vi "Integer Representation Test.vi"() -> ()   [LabVIEW 2026, in "Utility.lvlib"]
uses:
  Utility.lvlib
  Types/Signed Representation.ctl
  913b890a-b0f4-4715-82c4-53c9b125f797.vi
  de269a94-3f4e-4f39-b3db-9fb101915407.vi
  9b4d6897-da67-4ca5-9ae3-ea53d4320284.vi
  3e9a7e41-c2e1-426e-9bc1-8a394e217d85.vi
  1327767c-dc11-4062-be7d-752ab4d70a8a.vi
  1d7e0380-15ec-4017-ad21-249a48283e6f.vi
  7fe95ae4-1eaf-41d9-8065-e14043517ae9.vi
  1beec93f-fbc7-42dc-88dc-d3ecba0fc0bd.vi
  913b890a-b0f4-4715-82c4-53c9b125f797.vi/fdd2035b-52a6-4314-93d5-e6d0012ea0d5.vi
  913b890a-b0f4-4715-82c4-53c9b125f797.vi/d7ddfa2c-0539-47bf-9b9d-3a470632982d.vi
  913b890a-b0f4-4715-82c4-53c9b125f797.vi/b8120071-ec88-4802-9c07-9d147ec9c255.vi
  913b890a-b0f4-4715-82c4-53c9b125f797.vi/96d3ddf9-193f-4353-8b9f-7b29ff2119cb.vi
  913b890a-b0f4-4715-82c4-53c9b125f797.vi/a2043324-c5a4-4327-a6d6-ab77c0f4b7eb.vi
  de269a94-3f4e-4f39-b3db-9fb101915407.vi/075529c4-3756-4c35-a727-d79a570b4e4b.vi
  de269a94-3f4e-4f39-b3db-9fb101915407.vi/f2b159a7-3f15-4c07-8087-86d897f3e084.vi
  de269a94-3f4e-4f39-b3db-9fb101915407.vi/e7f4747e-5a28-4a2e-9592-f11bd74c8d05.vi
  de269a94-3f4e-4f39-b3db-9fb101915407.vi/dfb42b1f-79ab-4f7c-b389-1108b947dcfb.vi
  de269a94-3f4e-4f39-b3db-9fb101915407.vi/5f52ec6b-8d9c-4a1b-8cba-4e2f2acbbc65.vi
  de269a94-3f4e-4f39-b3db-9fb101915407.vi/9402299f-8d08-4b56-b955-c752433d99a7.vi
  de269a94-3f4e-4f39-b3db-9fb101915407.vi/587ca7da-2917-4b98-b856-e292118fa9d0.vi
  de269a94-3f4e-4f39-b3db-9fb101915407.vi/d9cf77ad-bfa9-4690-bb58-8188d63c027f.vi
  de269a94-3f4e-4f39-b3db-9fb101915407.vi/0dbe1b4e-815d-48eb-bf8e-9c4112dc030e.vi
  9b4d6897-da67-4ca5-9ae3-ea53d4320284.vi/fdd2035b-52a6-4314-93d5-e6d0012ea0d5.vi
  9b4d6897-da67-4ca5-9ae3-ea53d4320284.vi/d7ddfa2c-0539-47bf-9b9d-3a470632982d.vi
  9b4d6897-da67-4ca5-9ae3-ea53d4320284.vi/b8120071-ec88-4802-9c07-9d147ec9c255.vi
  9b4d6897-da67-4ca5-9ae3-ea53d4320284.vi/96d3ddf9-193f-4353-8b9f-7b29ff2119cb.vi
  9b4d6897-da67-4ca5-9ae3-ea53d4320284.vi/a2043324-c5a4-4327-a6d6-ab77c0f4b7eb.vi
  3e9a7e41-c2e1-426e-9bc1-8a394e217d85.vi/075529c4-3756-4c35-a727-d79a570b4e4b.vi
  3e9a7e41-c2e1-426e-9bc1-8a394e217d85.vi/f2b159a7-3f15-4c07-8087-86d897f3e084.vi
  3e9a7e41-c2e1-426e-9bc1-8a394e217d85.vi/e7f4747e-5a28-4a2e-9592-f11bd74c8d05.vi
  3e9a7e41-c2e1-426e-9bc1-8a394e217d85.vi/dfb42b1f-79ab-4f7c-b389-1108b947dcfb.vi
  3e9a7e41-c2e1-426e-9bc1-8a394e217d85.vi/5f52ec6b-8d9c-4a1b-8cba-4e2f2acbbc65.vi
  3e9a7e41-c2e1-426e-9bc1-8a394e217d85.vi/9402299f-8d08-4b56-b955-c752433d99a7.vi
  3e9a7e41-c2e1-426e-9bc1-8a394e217d85.vi/587ca7da-2917-4b98-b856-e292118fa9d0.vi
  3e9a7e41-c2e1-426e-9bc1-8a394e217d85.vi/d9cf77ad-bfa9-4690-bb58-8188d63c027f.vi
  3e9a7e41-c2e1-426e-9bc1-8a394e217d85.vi/0dbe1b4e-815d-48eb-bf8e-9c4112dc030e.vi
  1327767c-dc11-4062-be7d-752ab4d70a8a.vi/fdd2035b-52a6-4314-93d5-e6d0012ea0d5.vi
  1327767c-dc11-4062-be7d-752ab4d70a8a.vi/d7ddfa2c-0539-47bf-9b9d-3a470632982d.vi
  1327767c-dc11-4062-be7d-752ab4d70a8a.vi/b8120071-ec88-4802-9c07-9d147ec9c255.vi
  1327767c-dc11-4062-be7d-752ab4d70a8a.vi/96d3ddf9-193f-4353-8b9f-7b29ff2119cb.vi
  1327767c-dc11-4062-be7d-752ab4d70a8a.vi/a2043324-c5a4-4327-a6d6-ab77c0f4b7eb.vi
  1d7e0380-15ec-4017-ad21-249a48283e6f.vi/075529c4-3756-4c35-a727-d79a570b4e4b.vi
  1d7e0380-15ec-4017-ad21-249a48283e6f.vi/f2b159a7-3f15-4c07-8087-86d897f3e084.vi
  1d7e0380-15ec-4017-ad21-249a48283e6f.vi/e7f4747e-5a28-4a2e-9592-f11bd74c8d05.vi
  1d7e0380-15ec-4017-ad21-249a48283e6f.vi/dfb42b1f-79ab-4f7c-b389-1108b947dcfb.vi
  1d7e0380-15ec-4017-ad21-249a48283e6f.vi/5f52ec6b-8d9c-4a1b-8cba-4e2f2acbbc65.vi
  1d7e0380-15ec-4017-ad21-249a48283e6f.vi/9402299f-8d08-4b56-b955-c752433d99a7.vi
  1d7e0380-15ec-4017-ad21-249a48283e6f.vi/587ca7da-2917-4b98-b856-e292118fa9d0.vi
  1d7e0380-15ec-4017-ad21-249a48283e6f.vi/d9cf77ad-bfa9-4690-bb58-8188d63c027f.vi
  1d7e0380-15ec-4017-ad21-249a48283e6f.vi/0dbe1b4e-815d-48eb-bf8e-9c4112dc030e.vi
  7fe95ae4-1eaf-41d9-8065-e14043517ae9.vi/fdd2035b-52a6-4314-93d5-e6d0012ea0d5.vi
  7fe95ae4-1eaf-41d9-8065-e14043517ae9.vi/d7ddfa2c-0539-47bf-9b9d-3a470632982d.vi
  7fe95ae4-1eaf-41d9-8065-e14043517ae9.vi/b8120071-ec88-4802-9c07-9d147ec9c255.vi
  7fe95ae4-1eaf-41d9-8065-e14043517ae9.vi/96d3ddf9-193f-4353-8b9f-7b29ff2119cb.vi
  7fe95ae4-1eaf-41d9-8065-e14043517ae9.vi/a2043324-c5a4-4327-a6d6-ab77c0f4b7eb.vi
  1beec93f-fbc7-42dc-88dc-d3ecba0fc0bd.vi/075529c4-3756-4c35-a727-d79a570b4e4b.vi
  1beec93f-fbc7-42dc-88dc-d3ecba0fc0bd.vi/f2b159a7-3f15-4c07-8087-86d897f3e084.vi
  1beec93f-fbc7-42dc-88dc-d3ecba0fc0bd.vi/e7f4747e-5a28-4a2e-9592-f11bd74c8d05.vi
  1beec93f-fbc7-42dc-88dc-d3ecba0fc0bd.vi/dfb42b1f-79ab-4f7c-b389-1108b947dcfb.vi
  1beec93f-fbc7-42dc-88dc-d3ecba0fc0bd.vi/5f52ec6b-8d9c-4a1b-8cba-4e2f2acbbc65.vi
  1beec93f-fbc7-42dc-88dc-d3ecba0fc0bd.vi/9402299f-8d08-4b56-b955-c752433d99a7.vi
  1beec93f-fbc7-42dc-88dc-d3ecba0fc0bd.vi/587ca7da-2917-4b98-b856-e292118fa9d0.vi
  1beec93f-fbc7-42dc-88dc-d3ecba0fc0bd.vi/d9cf77ad-bfa9-4690-bb58-8188d63c027f.vi
  1beec93f-fbc7-42dc-88dc-d3ecba0fc0bd.vi/0dbe1b4e-815d-48eb-bf8e-9c4112dc030e.vi
  913b890a-b0f4-4715-82c4-53c9b125f797.vi/b8120071-ec88-4802-9c07-9d147ec9c255.vi/8ccb98a6-deb9-4b5a-be05-054c1c212d54.vi
  913b890a-b0f4-4715-82c4-53c9b125f797.vi/b8120071-ec88-4802-9c07-9d147ec9c255.vi/f171c548-4dcc-4c0c-949b-fc0df33543c2.vi
  913b890a-b0f4-4715-82c4-53c9b125f797.vi/b8120071-ec88-4802-9c07-9d147ec9c255.vi/d8adcdbd-60f3-48f3-8f6a-253ba0c2f91d.vi
  913b890a-b0f4-4715-82c4-53c9b125f797.vi/b8120071-ec88-4802-9c07-9d147ec9c255.vi/e61c01d5-f4be-4974-af39-63853a8697d8.vi
  913b890a-b0f4-4715-82c4-53c9b125f797.vi/96d3ddf9-193f-4353-8b9f-7b29ff2119cb.vi/8ccb98a6-deb9-4b5a-be05-054c1c212d54.vi
  913b890a-b0f4-4715-82c4-53c9b125f797.vi/96d3ddf9-193f-4353-8b9f-7b29ff2119cb.vi/f171c548-4dcc-4c0c-949b-fc0df33543c2.vi
  913b890a-b0f4-4715-82c4-53c9b125f797.vi/96d3ddf9-193f-4353-8b9f-7b29ff2119cb.vi/d8adcdbd-60f3-48f3-8f6a-253ba0c2f91d.vi
  913b890a-b0f4-4715-82c4-53c9b125f797.vi/96d3ddf9-193f-4353-8b9f-7b29ff2119cb.vi/e61c01d5-f4be-4974-af39-63853a8697d8.vi
  9b4d6897-da67-4ca5-9ae3-ea53d4320284.vi/b8120071-ec88-4802-9c07-9d147ec9c255.vi/8ccb98a6-deb9-4b5a-be05-054c1c212d54.vi
  9b4d6897-da67-4ca5-9ae3-ea53d4320284.vi/b8120071-ec88-4802-9c07-9d147ec9c255.vi/f171c548-4dcc-4c0c-949b-fc0df33543c2.vi
  9b4d6897-da67-4ca5-9ae3-ea53d4320284.vi/b8120071-ec88-4802-9c07-9d147ec9c255.vi/d8adcdbd-60f3-48f3-8f6a-253ba0c2f91d.vi
  9b4d6897-da67-4ca5-9ae3-ea53d4320284.vi/b8120071-ec88-4802-9c07-9d147ec9c255.vi/e61c01d5-f4be-4974-af39-63853a8697d8.vi
  9b4d6897-da67-4ca5-9ae3-ea53d4320284.vi/96d3ddf9-193f-4353-8b9f-7b29ff2119cb.vi/8ccb98a6-deb9-4b5a-be05-054c1c212d54.vi
  9b4d6897-da67-4ca5-9ae3-ea53d4320284.vi/96d3ddf9-193f-4353-8b9f-7b29ff2119cb.vi/f171c548-4dcc-4c0c-949b-fc0df33543c2.vi
  9b4d6897-da67-4ca5-9ae3-ea53d4320284.vi/96d3ddf9-193f-4353-8b9f-7b29ff2119cb.vi/d8adcdbd-60f3-48f3-8f6a-253ba0c2f91d.vi
  9b4d6897-da67-4ca5-9ae3-ea53d4320284.vi/96d3ddf9-193f-4353-8b9f-7b29ff2119cb.vi/e61c01d5-f4be-4974-af39-63853a8697d8.vi
  1327767c-dc11-4062-be7d-752ab4d70a8a.vi/b8120071-ec88-4802-9c07-9d147ec9c255.vi/8ccb98a6-deb9-4b5a-be05-054c1c212d54.vi
  1327767c-dc11-4062-be7d-752ab4d70a8a.vi/b8120071-ec88-4802-9c07-9d147ec9c255.vi/f171c548-4dcc-4c0c-949b-fc0df33543c2.vi
  1327767c-dc11-4062-be7d-752ab4d70a8a.vi/b8120071-ec88-4802-9c07-9d147ec9c255.vi/d8adcdbd-60f3-48f3-8f6a-253ba0c2f91d.vi
  1327767c-dc11-4062-be7d-752ab4d70a8a.vi/b8120071-ec88-4802-9c07-9d147ec9c255.vi/e61c01d5-f4be-4974-af39-63853a8697d8.vi
  1327767c-dc11-4062-be7d-752ab4d70a8a.vi/96d3ddf9-193f-4353-8b9f-7b29ff2119cb.vi/8ccb98a6-deb9-4b5a-be05-054c1c212d54.vi
  1327767c-dc11-4062-be7d-752ab4d70a8a.vi/96d3ddf9-193f-4353-8b9f-7b29ff2119cb.vi/f171c548-4dcc-4c0c-949b-fc0df33543c2.vi
  1327767c-dc11-4062-be7d-752ab4d70a8a.vi/96d3ddf9-193f-4353-8b9f-7b29ff2119cb.vi/d8adcdbd-60f3-48f3-8f6a-253ba0c2f91d.vi
  1327767c-dc11-4062-be7d-752ab4d70a8a.vi/96d3ddf9-193f-4353-8b9f-7b29ff2119cb.vi/e61c01d5-f4be-4974-af39-63853a8697d8.vi
  7fe95ae4-1eaf-41d9-8065-e14043517ae9.vi/b8120071-ec88-4802-9c07-9d147ec9c255.vi/8ccb98a6-deb9-4b5a-be05-054c1c212d54.vi
  7fe95ae4-1eaf-41d9-8065-e14043517ae9.vi/b8120071-ec88-4802-9c07-9d147ec9c255.vi/f171c548-4dcc-4c0c-949b-fc0df33543c2.vi
  7fe95ae4-1eaf-41d9-8065-e14043517ae9.vi/b8120071-ec88-4802-9c07-9d147ec9c255.vi/d8adcdbd-60f3-48f3-8f6a-253ba0c2f91d.vi
  7fe95ae4-1eaf-41d9-8065-e14043517ae9.vi/b8120071-ec88-4802-9c07-9d147ec9c255.vi/e61c01d5-f4be-4974-af39-63853a8697d8.vi
  7fe95ae4-1eaf-41d9-8065-e14043517ae9.vi/96d3ddf9-193f-4353-8b9f-7b29ff2119cb.vi/8ccb98a6-deb9-4b5a-be05-054c1c212d54.vi
  7fe95ae4-1eaf-41d9-8065-e14043517ae9.vi/96d3ddf9-193f-4353-8b9f-7b29ff2119cb.vi/f171c548-4dcc-4c0c-949b-fc0df33543c2.vi
  7fe95ae4-1eaf-41d9-8065-e14043517ae9.vi/96d3ddf9-193f-4353-8b9f-7b29ff2119cb.vi/d8adcdbd-60f3-48f3-8f6a-253ba0c2f91d.vi
  7fe95ae4-1eaf-41d9-8065-e14043517ae9.vi/96d3ddf9-193f-4353-8b9f-7b29ff2119cb.vi/e61c01d5-f4be-4974-af39-63853a8697d8.vi
panel:
  out "Equal?":bool
  out "Equal?":bool
  out "I8 Value":i8
  out "I16 Value":i16
  out "Equal?":bool
  out "I32 Value out":i32
  out "Equal?":bool
  out "I64 Value out":i64
  out "Valid?":bool=TRUE
  out "Valid?":bool=TRUE
  out "Valid?":bool=TRUE
  out "Valid?":bool=TRUE
  out "U8 Value":u8 format="%02x"
  out "U16 Value":u16 format="%04x"
  out "U64 Value":u64 format="%016x"
  out "U32 Value":u32 format="%08x"
  out "I8 Value":i8
  out "I16 Value":i16
  in  "I64 Value":i64
  in  "Signed representation":T1
  out "I32 Value":i32
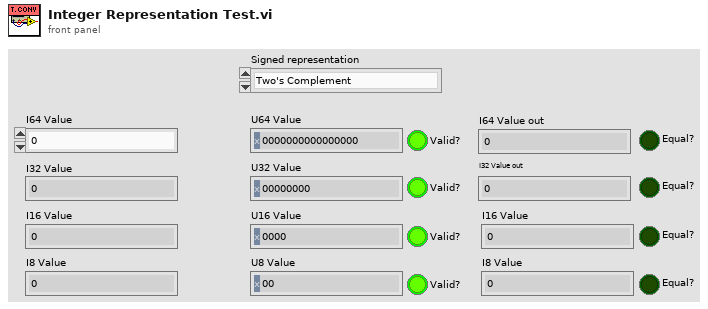
[diagram p1: front panel]
types:
  T1 = typedef "Utility.lvlib/Signed Representation.ctl" = enum16{"Two's Complement", "Offset Binary", "Sign-Magnitude", "Ones' Complement"}
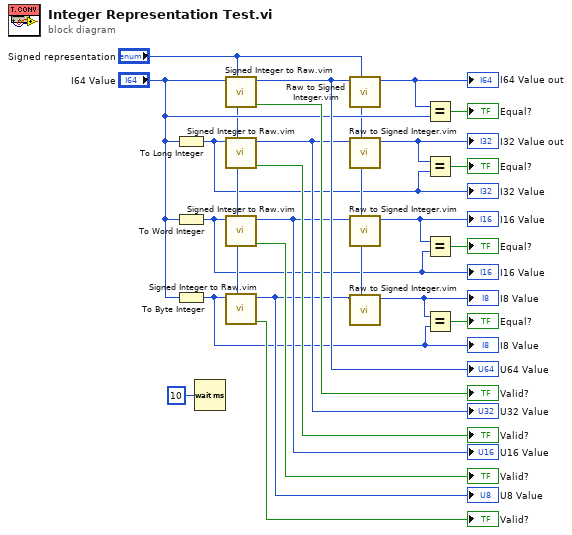
[diagram p0: block diagram]
diagram:
  n1 = To Long Integer(number="I64 Value") -> (32bit integer=w8:i32)
  "I32 Value" <- w8
  n2 = To Word Integer(number="I64 Value") -> (16bit integer=w4:i16)
  "I16 Value" <- w4
  n3 = To Byte Integer(number="I64 Value") -> (8bit integer=w1:i8)
  "I8 Value" <- w1
  n4 = Wait (ms)(milliseconds to wait=u32 10) -> ()  [unwired: 1 out]
  n5 = call "Signed Integer to Raw.vim"("Signed representation"="Signed representation", "Value in"="I64 Value") -> ("Valid?"=→"Valid?":bool, "Value (raw)"=w18:u64)  [unwired: 8 in]
  "U64 Value" <- w18
  n6 = call "Signed Integer to Raw.vim"("Signed representation"="Signed representation", "Value in"=w8) -> ("Valid?"=→"Valid?":bool, "Value (raw)"=w12:u32)  [unwired: 8 in]
  "U32 Value" <- w12
  n7 = call "Signed Integer to Raw.vim"("Signed representation"="Signed representation", "Value in"=w4) -> ("Valid?"=→"Valid?":bool, "Value (raw)"=w11:u16)  [unwired: 8 in]
  "U16 Value" <- w11
  n8 = call "Signed Integer to Raw.vim"("Signed representation"="Signed representation", "Value in"=w1) -> ("Valid?"=→"Valid?":bool, "Value (raw)"=w7:u8)  [unwired: 8 in]
  "U8 Value" <- w7
  n9 = call "Raw to Signed Integer.vim"("Signed representation"="Signed representation", "Value (raw)"=w18) -> ("Value out"=w17:i64)  [unwired: 8 in, 1 out]
  "I64 Value out" <- w17
  n10 = call "Raw to Signed Integer.vim"("Signed representation"="Signed representation", "Value (raw)"=w12) -> ("Value out"=w9:i32)  [unwired: 8 in, 1 out]
  "I32 Value out" <- w9
  n11 = call "Raw to Signed Integer.vim"("Signed representation"="Signed representation", "Value (raw)"=w11) -> ("Value out"=w5:i16)  [unwired: 8 in, 1 out]
  "I16 Value" <- w5
  n12 = call "Raw to Signed Integer.vim"("Signed representation"="Signed representation", "Value (raw)"=w7) -> ("Value out"=w2:i8)  [unwired: 8 in, 1 out]
  "I8 Value" <- w2
  n13 = Equal?(x=w17, y="I64 Value") -> (x = y?=→"Equal?":bool)
  n14 = Equal?(x=w9, y=w8) -> (x = y?=→"Equal?":bool)
  n15 = Equal?(x=w5, y=w4) -> (x = y?=→"Equal?":bool)
  n16 = Equal?(x=w2, y=w1) -> (x = y?=→"Equal?":bool)
